vi "Check_The_Current_Profile.vi"(8 "error in (no error) 2":errorcluster) -> (0 "error in (no error) 3":errorcluster, 1 "Test Type":string, 2 "path":path, 3 "?":string, 5 "Enum":T1)   [LabVIEW 2021]
uses:
  HI-POT_Driver/Hi-pot_Driver.ctl
  Control/Ini.ctl
panel:
  out "value":string
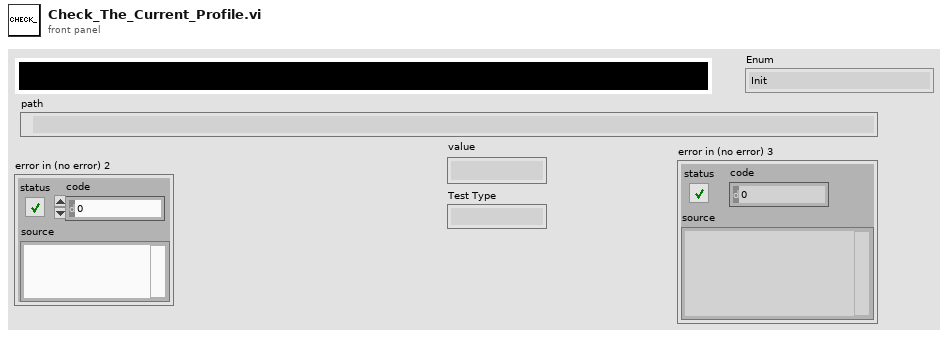
[diagram p1: front panel]
types:
  T1 = typedef "Hi-pot_Driver.ctl" = enum16{"Init ", "Interlock status", "Set UP DCW", "Set UP ACW", "Set UP IR", "Read", "Clear", "Close"}
  T2 = typedef "Ini.ctl" = enum16{"Write", "Read"}
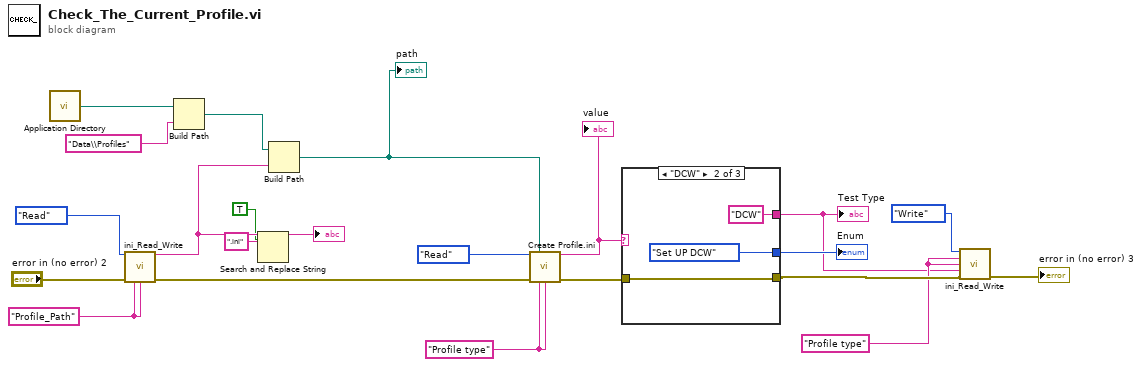
[diagram p0: block diagram]
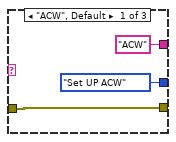
[diagram p2: hidden frame]
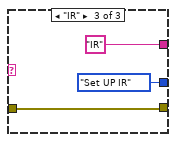
[diagram p3: hidden frame]
diagram:
  w10 = "Profile type" ("Write key")
  w14 = "Profile type" ("Write key")
  w21 = "Profile_Path" ("Read Section")
  n1 = call <vilib>:"Application Directory.vi"() -> ("Application Directory"=w8:path)
  n2 = call "ini_Read_Write.vi"(0:Ini."Read", "error in (no error) 2"="error in (no error) 2", "Read Section"=w21, "Read Key"=w21) -> ("value"=w5:string, "error in (no error) 3"=w17:errorcluster)  [unwired: 10 in]
  n3 = Build Path(base path=w8, name or relative path="Data\\Profiles" ("Read Section")) -> (appended path=w6:path)
  n4 = Search and Replace String(replace all?=TRUE ("replace all? (F)"), input string=w5, search string=".ini") -> (result string=→"?":string)  [unwired: 5 in, 3 out]
  n5 = Build Path(base path=w6, name or relative path=w5) -> (appended path=w1:path)
  "path" <- w1
  n6 = call "Create Profile.ini.vi"(0:Ini."Read", "configuration file path"=w1, "error in (no error)"=w17, "Read Section"=w14, "Read Key"=w14) -> ("value"=w15:string, "error in (no error) 3"=w16:errorcluster)  [unwired: 9 in]
  "value" <- w15
  n7 = case shown="\"DCW\"" w15 {
    tunnel: w16 -> [w25 w27 w31]
    tunnel: [w25 w27 w31] -> w12
    tunnel: [Hi-pot_Driver."Set UP ACW" Hi-pot_Driver."Set UP DCW" Hi-pot_Driver."Set UP IR"] -> w19
    tunnel: ["ACW" "DCW" "IR"] -> w9
    frame "ACW", Default {
    }
    frame "DCW" {
    }
    frame "IR" {
    }
  }
  "Enum" <- w19
  "Test Type" <- w9
  n8 = call "ini_Read_Write.vi"(0:Ini."Write", "Write Section"=w10, "Write key"=w10, "Write"=w9, "error in (no error) 2"=w12) -> ("error in (no error) 3"=→"error in (no error) 3":errorcluster)  [unwired: 9 in, 1 out]
